vi "Write Generated files.vi"(9 "ProjectItem in":refnum<class "ProjectItem.lvclass">, 10 "Generated files":path[](array[path]), 11 "BuildManager in":refnum<class "BuildManager.lvclass">) -> (3 "BuildManager out":refnum<class "BuildManager.lvclass">)   [LabVIEW 2019, in "SolutionBuilder.lvlib" / "BuildManager.lvclass"]
uses:
  BuildManager.lvclass
  ProjectItem/ProjectItem.lvclass
  ProjectItem/ProjectItem.lvclass/ProjectItem.ctl
  BuildManager.lvclass/BuildManager.ctl
  BuildProjectInfo.ctl
  <vilib>/Utility/miscctls.llb/LVMapReplaceAction.ctl
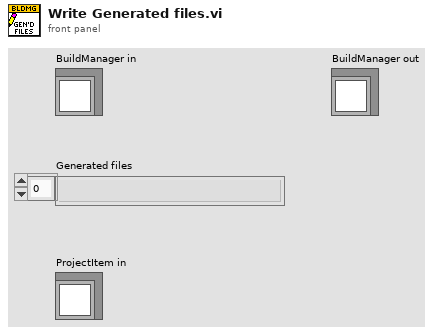
[diagram p1: front panel]
types:
  T1 = typedef "SolutionBuilder.lvlib/BuildManager.lvclass/BuildProjectInfo.ctl" = cluster{"Project path":string, "Build spec name":string, "Target":string, "Version string":string}
  T2 = typedef "LVMapReplaceAction.ctl" = enum32{"Modify Entry only if found", "Add or Modify Entry", "Delete Entry"}
  T3 = typedef "SolutionBuilder.lvlib/BuildManager.lvclass/GeneratedFile.ctl" = map{T1, set{string}}
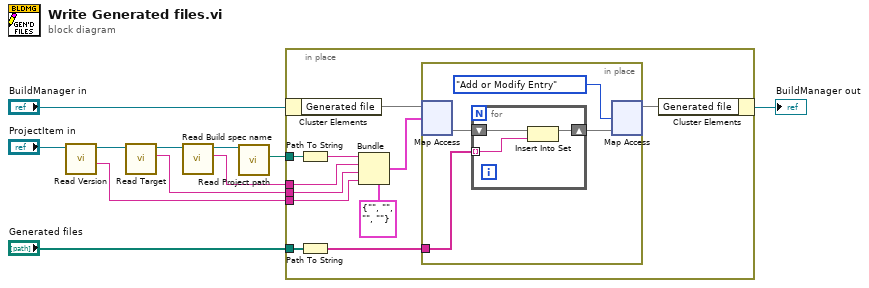
[diagram p0: block diagram]
diagram:
  n1 = call "Read Version.vi"("ProjectItem in"="ProjectItem in") -> ("Version string"=w1:string, "ProjectItem out"=w2:refnum<class "ProjectItem.lvclass">)  [unwired: 8 in, 1 out]
  n2 = call "Read Target.vi"("ProjectItem in"=w2) -> ("Target"=w4:string, "ProjectItem out"=w5:refnum<class "ProjectItem.lvclass">)  [unwired: 9 in]
  n3 = call "Read Build spec name.vi"("ProjectItem in"=w5) -> ("Build spec name"=w9:string, "ProjectItem out"=w10:refnum<class "ProjectItem.lvclass">)  [unwired: 9 in]
  n4 = call "Read Project path.vi"("ProjectItem in"=w10) -> ("Project path"=w8:path)  [unwired: 9 in, 1 out]
  n5 = in-place {
    in-place-border: "Generated files" -> [w15]
    in-place-border: w9 -> [w22]
    in-place-border: w8 -> [w21]
    in-place-border: w4 -> [w14]
    in-place-border: w1 -> [w12]
    n6 = in-place-cluster #1("BuildManager in") -> ("Generated file"=w20:T3)
    n7 = Path To String(path=w21) -> (string=w17:string)
    n8 = Path To String(path=w15) -> (string=w16:string[])
    n9 = Bundle(cluster=T1 {"Project path"="", "Build spec name"="", "Target"="", "Version string"=""} ("Parent info"), "Project path"=w17, "Build spec name"=w22, "Target"=w14, "Version string"=w12) -> (w18:T1)
    n10 = in-place {
      in-place-border: w16 -> [w24]
      n11 = in-place-map #2(w20, w18) -> (w26:set{string})  [unwired: 1 in, 1 out]
      n12 = for {
        shift-right: [w27] -> w25
        shift-left: w26 -> [w29]
        tunnel: w24 -> [w28] mode=indexing
        n13 = Insert Into Set(10:w28, 11:w29) -> (3:w27:set{string})  [unwired: 1 out]
      }
      n14 = in-place-map #2(w25, LVMapReplaceAction."Add or Modify Entry" ("action")) -> (w19:T3)  [unwired: 2 out]
    }
    n15 = in-place-cluster #1("Generated file"=w19) -> (→"BuildManager out":refnum<class "BuildManager.lvclass">)
  }
